vi "mainOCR _PC.vi"() -> ()   [LabVIEW 2025]
uses:
  ocr/ocr.lvclass
  <vilib>/vision/Image Controls.llb/IMAQ Image.ctl
panel:
  out "SetDevice":string
  out "uploadSucc":i32
  out "InitRecDec Success":string
  out "Numeric":i32
  out "Image":T1(plugin-control)
  in  "stop":bool
  in  "NEXT Button":bool
  in  "device":enum16{"CPU", "GPU0"}(ring)
  in  "PathImage 2":path=path "D:/Test/dllTest/images_2"
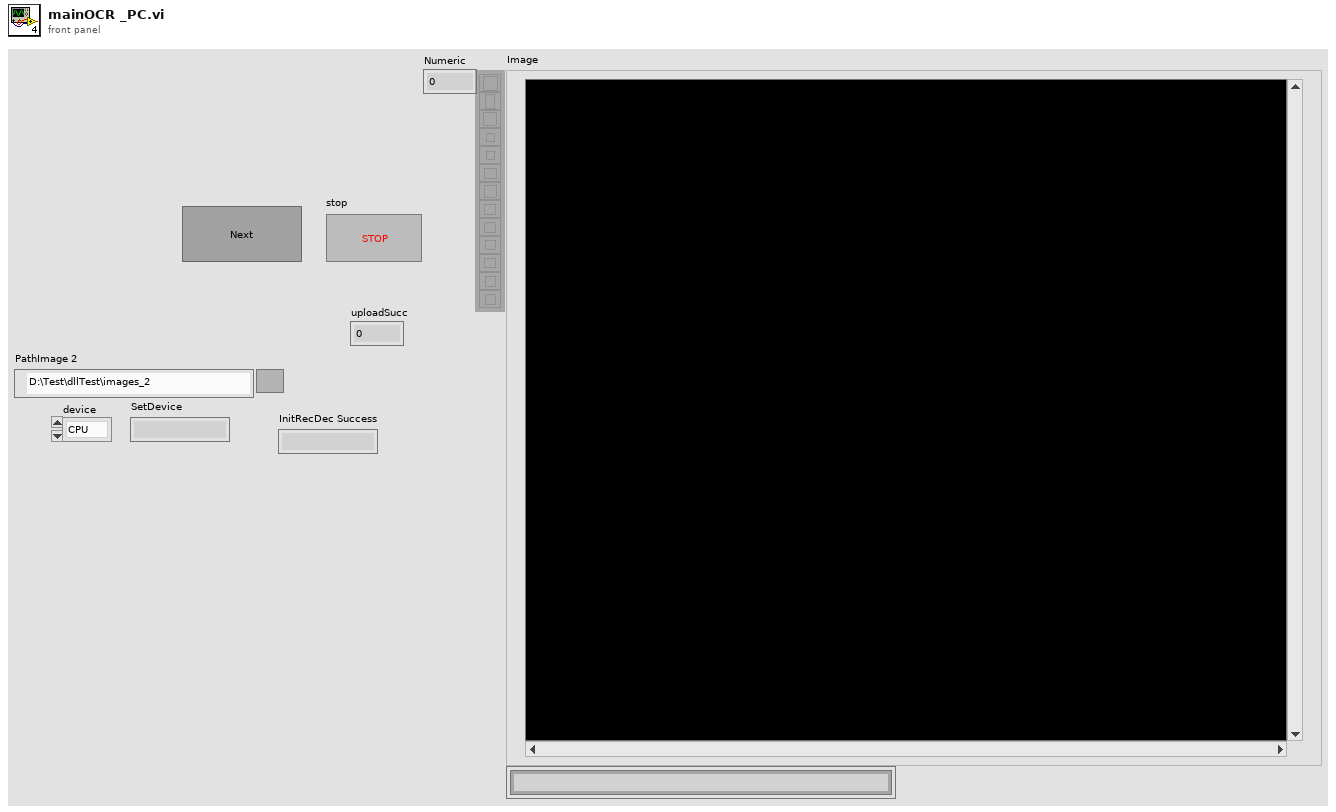
[diagram p1: front panel]
types:
  T1 = typedef "IMAQ Image.ctl" = refnum<image>
  T2 = typedef "adsOCR.lvlib/ocr.lvclass/TextDecRecResult2L.ctl" = cluster{"imgIdx":i32, "TLx":i32, "TLy":i32, "BRx":i32, "BRy":i32, "angle":sgl, "txtLen":i32}
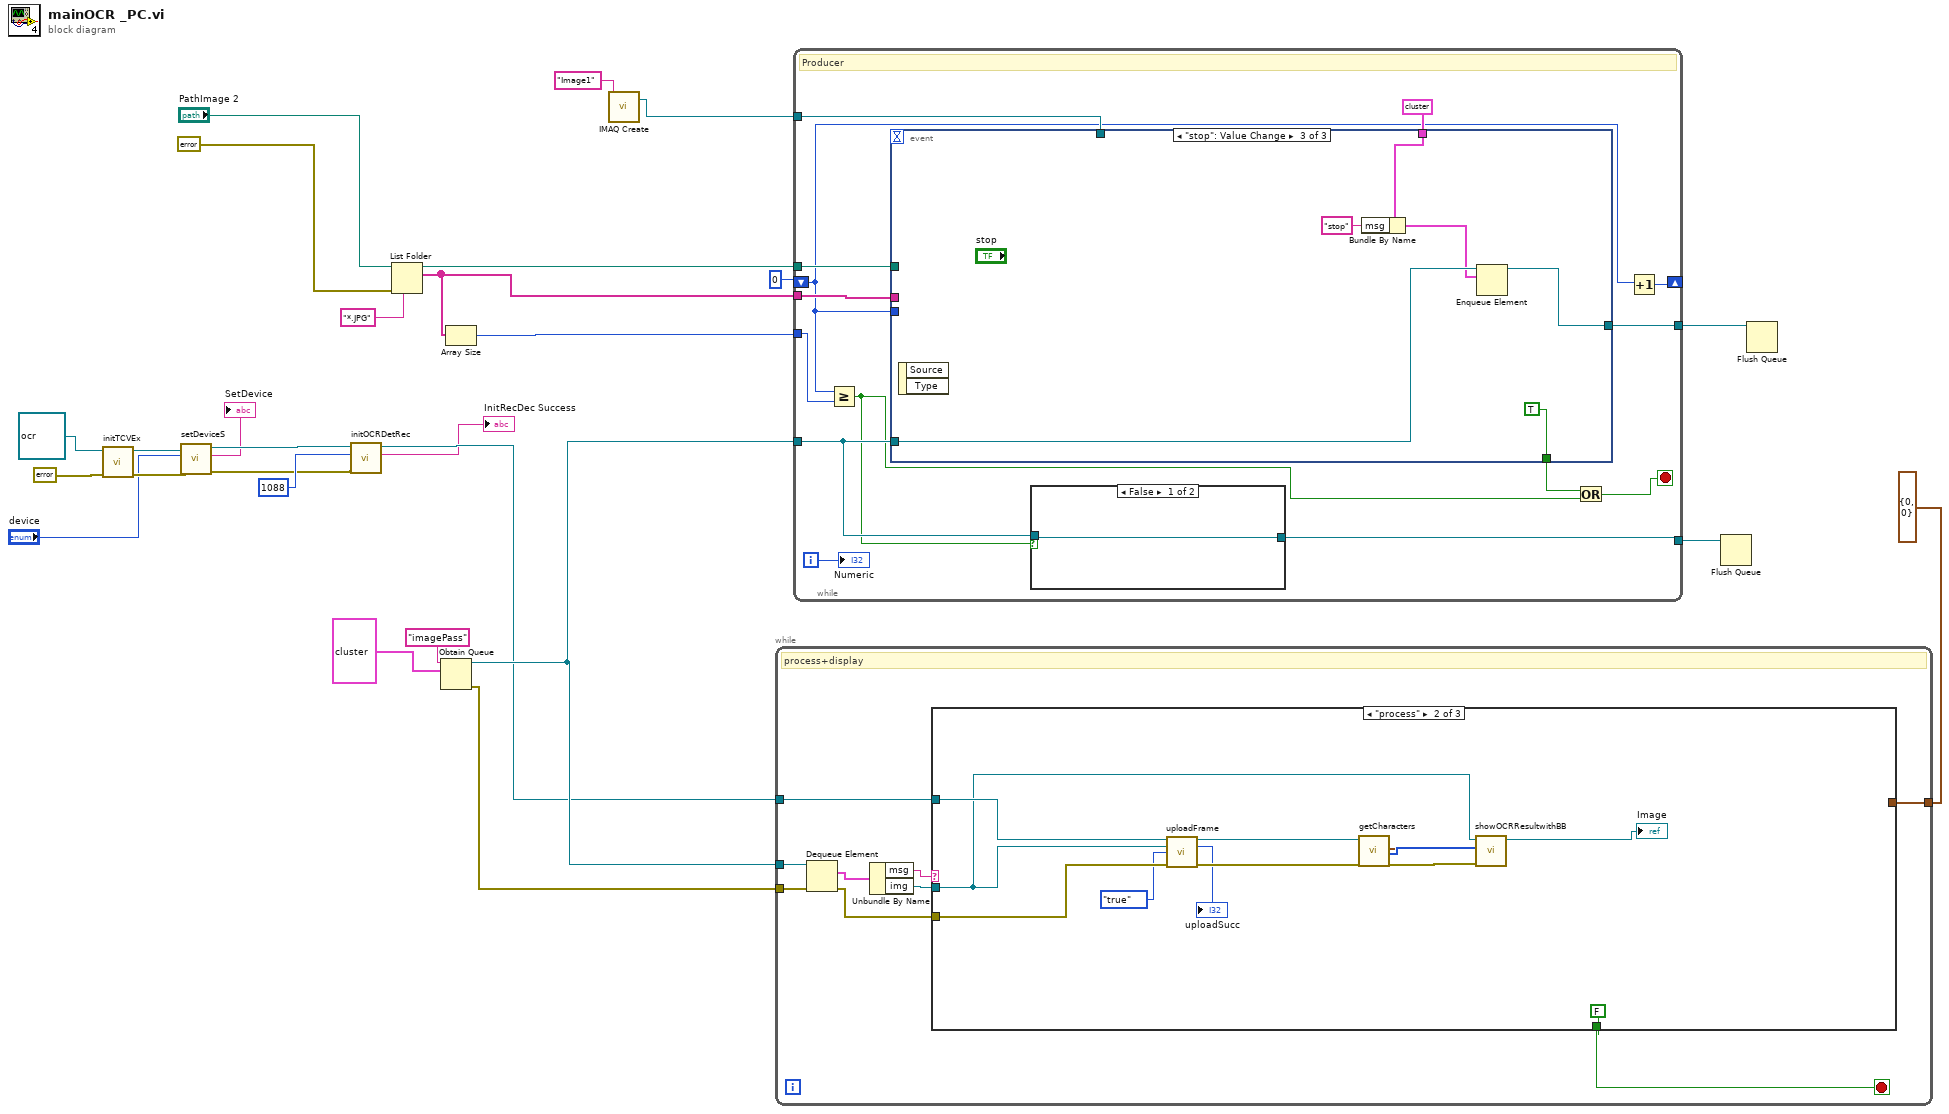
[diagram p0: block diagram]
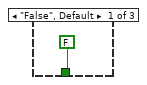
[diagram p2: hidden frame]
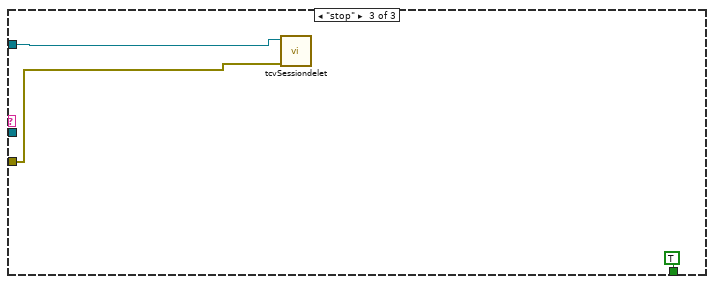
[diagram p3: hidden frame]
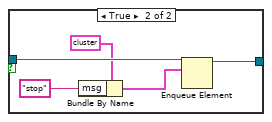
[diagram p4: hidden frame]
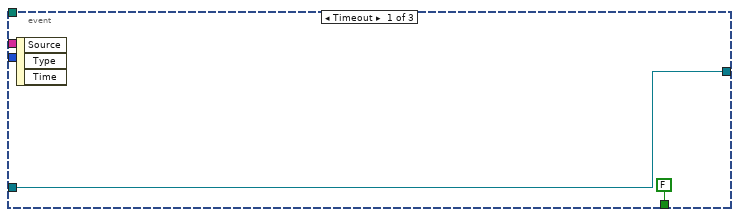
[diagram p5: hidden frame]
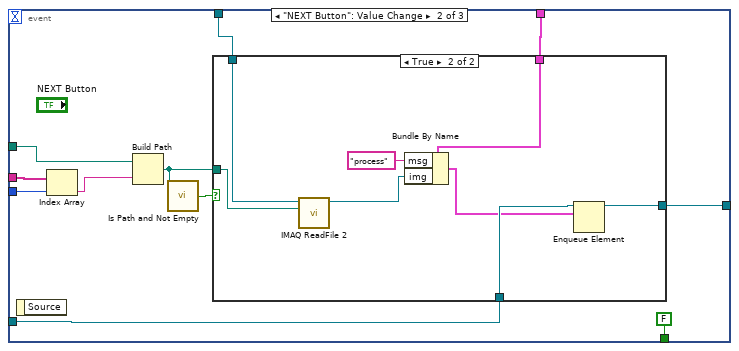
[diagram p6: hidden frame]
diagram:
  n1 = call-dynamic "initTCVEx.vi"("error in (no error)"=errorcluster {"status"=FALSE, "code"=0, "source"=""}, "tcv in"=refnum<class "ocr.lvclass"> refnum ("ocr in")) -> ("error out"=w22:errorcluster, "tcv out"=w23:refnum<class "ocr.lvclass">)  [unwired: 8 in]
  n2 = call-dynamic "setDeviceS.vi"("error in (no error)"=w22, "devices"="device", "tcv in"=w23) -> ("error out"=w3:errorcluster, "SetDevice"=→"SetDevice":string, "tcv out"=w6:refnum<class "ocr.lvclass">)  [unwired: 6 in]
  n3 = call "initOCRDetRec.vi"("error in (no error)"=w3, "targetSize"=1088, "tcv in"=w6) -> ("InitRecDec Success"=→"InitRecDec Success":string, "ocr out"=w5:refnum<class "ocr.lvclass">)  [unwired: 5 in, 2 out]
  n4 = List Folder(path="PathImage 2", pattern="*.JPG", error in=errorcluster {"status"=FALSE, "code"=0, "source"=""}) -> (path out=w19:path, filenames=w11:string[])  [unwired: 1 in, 2 out]
  n5 = Obtain Queue(name (unnamed)="imagePass", element data type=cluster{"msg":string, "img":T1} {"msg"="", "img"=refnum}) -> (queue out=w12:refnum<queue>, error out=w9:errorcluster)  [unwired: 3 in, 1 out]
  n6 = Array Size(array=w11) -> (size(s)=w17:i32)
  n7 = call "IMAQ Create"("Image Name"="Image1") -> ("New Image"=w15:T1)  [unwired: 4 in, 1 out]
  n8 = while {
    tunnel: cluster{"x":i32, "y":i32} {"x"=0, "y"=0} -> [w31]
    tunnel: w12 -> [w36]
    tunnel: w5 -> [w32]
    tunnel: w9 -> [w29]
    stop <- w30 stop-if-true
    # "process+display"
    n9 = Dequeue Element(queue=w36, error in (no error)=w29) -> (element=w35:cluster{"msg":string, "img":T1}, error out=w28:errorcluster)  [unwired: 1 in, 2 out]
    n10 = Unbundle By Name(w35) -> ("msg"=w34:string, "img"=w33:T1)
    n11 = case shown="\"process\"" w34 {
      tunnel: w33 -> [_ w43 _]
      tunnel: w32 -> [_ w48 w51]
      tunnel: w31 -> [_ _ _]
      tunnel: [FALSE FALSE TRUE] -> w30
      tunnel: w28 -> [_ w46 w50]
      frame "False", Default {
      }
      frame "process" {
        n12 = call-dynamic "uploadFrame.vi"("tcv in"=w48, "Image"=w43, "normalise"=enum32{"false", "true"}."true", "error in (no error)"=w46) -> ("tcv out"=w47:refnum<class "ocr.lvclass">, "uploadSucc"=→"uploadSucc":i32, "error out"=w44:errorcluster)  [unwired: 8 in, 1 out]
        n13 = call-dynamic "getCharacters.vi"("ocr in"=w47, "error in (no error)"=w44) -> ("TextDecRecResult2L"=w40:T2[], "chars"=w42:u8[], "error out"=w41:errorcluster)  [unwired: 12 in, 3 out]
        n14 = call "showOCRResultwithBB.vi"("error in"=w41, "Array"=w40, "chars"=w42, "Image in"=w43) -> ("Image out"=→"Image":T1)  [unwired: 6 in, 1 out]
      }
      frame "stop" {
        n15 = call-dynamic "tcvSessiondelet.vi"("error in (no error)"=w50, "tcv in"=w51) -> ()  [unwired: 8 in, 2 out]
      }
    }
  }
  n16 = while {
    shift-right: [w62] -> _
    shift-left: 0 -> [w54]
    tunnel: w19 -> [w66]
    tunnel: w11 -> [w65]
    tunnel: w17 -> [w64]
    tunnel: w15 -> [w63]
    tunnel: w12 -> [w57]
    tunnel: [w58] -> w8
    tunnel: [w55] -> w7
    i -> [w53]
    stop <- w59 stop-if-true
    # "Producer"
    n17 = Greater Or Equal?(x=w54, y=w64) -> (x >= y?=w56:bool)
    n18 = event shown="[2] \"stop\": Value Change" {
      selector: _ -> [_ _ _]
      dyn-events: _ -> [_ _ _]
      timeout: _ -> [_ _ _]
      tunnel: w66 -> [_ w85 _]
      tunnel: w65 -> [_ w82 _]
      tunnel: w63 -> [_ w84 _]
      tunnel: w57 -> [w73 w83 w98]
      tunnel: w54 -> [_ w81 _]
      tunnel: cluster{"msg":string, "img":T1} {"msg"="", "img"=refnum} -> [_ w77 w100]
      tunnel: [FALSE FALSE TRUE] -> w60
      tunnel: [w73 w75 w95] -> w58
      event Timeout {
        n19 = event-data() -> ()  [unwired: 1 in, 3 out]
      }
      event "NEXT Button": Value Change {
        n20 = event-data() -> ()  [unwired: 1 in, 1 out]
        n21 = Index Array(array=w82, index=w81) -> (element=w80:string)
        n22 = Build Path(base path=w85, name or relative path=w80) -> (appended path=w79:path)
        n23 = call <vilib>:"Is Path and Not Empty.vi"("path"=w79) -> ("Is Path and Not Empty?"=w78:bool)  [unwired: 4 in]
        n24 = case shown="True" w78 {
          tunnel: w84 -> [_ w94]
          tunnel: w79 -> [_ w93]
          tunnel: w83 -> [w86 w92]
          tunnel: w77 -> [_ w88]
          tunnel: [w86 w87] -> w75
          frame False {
          }
          frame True {
            n25 = call "IMAQ ReadFile 2"("File Path"=w93, "Image"=w94) -> ("Image Out"=w90:T1)  [unwired: 5 in, 4 out]
            n26 = Bundle By Name(cluster=w88, "msg"="process", "img"=w90) -> (w89:cluster{"msg":string, "img":T1})
            n27 = Enqueue Element(queue=w92, element=w89) -> (queue out=w87:refnum<queue>)  [unwired: 2 in, 2 out]
          }
        }
      }
      event "stop": Value Change {
        n28 = event-data() -> ()  [unwired: 1 in, 2 out]
        n29 = Bundle By Name(cluster=w100, "msg"="stop") -> (w97:cluster{"msg":string, "img":T1})
        n30 = Enqueue Element(queue=w98, element=w97) -> (queue out=w95:refnum<queue>)  [unwired: 2 in, 2 out]
      }
    }
    n31 = case shown="False" w56 {
      tunnel: w57 -> [w67 w71]
      tunnel: [w67 w68] -> w55
      frame False {
      }
      frame True {
        n32 = Bundle By Name(cluster=cluster{"msg":string, "img":T1} {"msg"="", "img"=refnum}, "msg"="stop") -> (w72:cluster{"msg":string, "img":T1})
        n33 = Enqueue Element(queue=w71, element=w72) -> (queue out=w68:refnum<queue>)  [unwired: 2 in, 2 out]
      }
    }
    n34 = Or(x=w60, y=w56) -> (x .or. y?=w59:bool)
    n35 = Increment(x=w54) -> (x+1=w62:i32)
    "Numeric" <- w53
  }
  n36 = Flush Queue(queue=w7) -> ()  [unwired: 1 in, 3 out]
  n37 = Flush Queue(queue=w8) -> ()  [unwired: 1 in, 3 out]
